vi "Read String.vi"(8 "error in (no error)":errorcluster, 11 "Event in":refnum<class "Event String.lvclass">) -> (0 "error out":errorcluster, 2 "String":string, 3 "Event out":refnum<class "Event String.lvclass">)   [LabVIEW 2023, in "MVC Actors.lvlib" / "Event String.lvclass"]
uses:
  Event String.lvclass
  Event String.lvclass/Event String.ctl
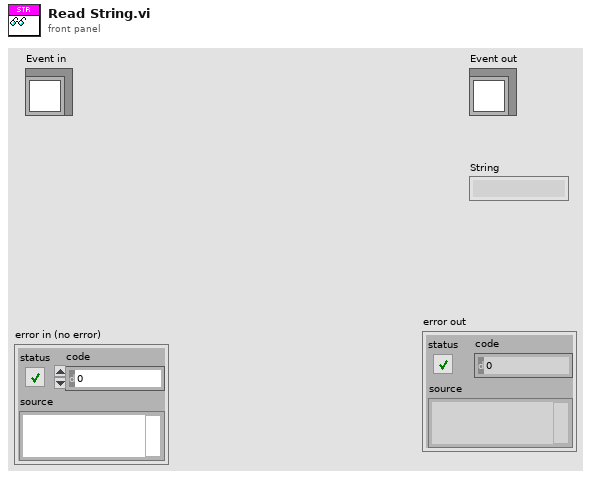
[diagram p1: front panel]
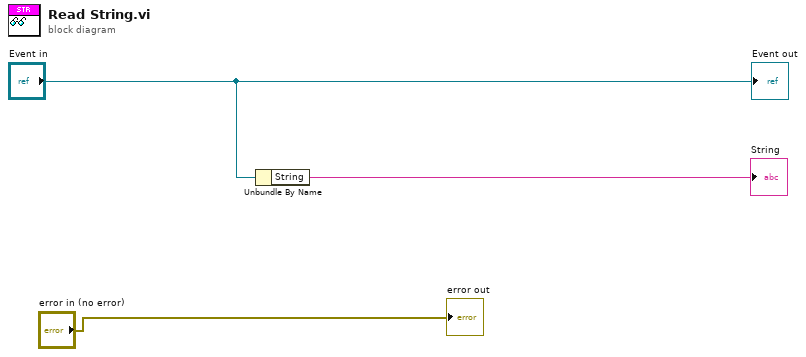
[diagram p0: block diagram]
diagram:
  n1 = Unbundle By Name("Event in") -> ("String"=→"String":string)
  "Event out" <- "Event in"
  "error out" <- "error in (no error)"
